vi "Read Configuration Name.vi"(8 "error in":errorcluster, 11 "PL_System Configuration in":refnum<class "PL_System Configuration.lvclass">) -> (0 "error out":errorcluster, 2 "Configuration Name":string, 3 "PL_System Configuration out":refnum<class "PL_System Configuration.lvclass">)   [LabVIEW 2013, in "PL_System Configuration.lvclass"]
uses:
  PL_System Configuration.lvclass
  <vilib>/NI/Configuration Framework/serializable configuration/NISE_CEF_serializable configuration.lvclass
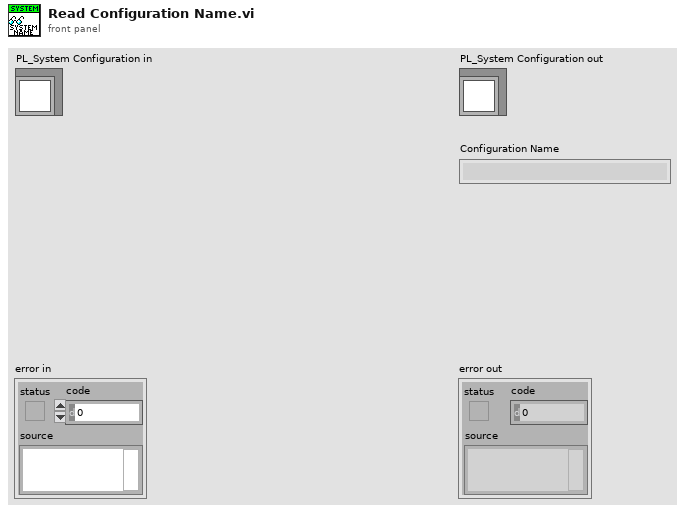
[diagram p1: front panel]
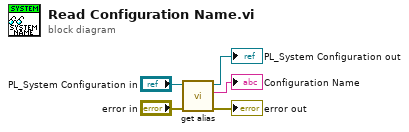
[diagram p0: block diagram]
diagram:
  n1 = call <vilib>:"get alias.vi"("error in"="error in", "configuration in"="PL_System Configuration in") -> ("error out"=→"error out":errorcluster, "alias"=→"Configuration Name":string, "configuration out"=→"PL_System Configuration out":refnum<class "PL_System Configuration.lvclass">)  [unwired: 7 in]
